vi "_LabeledRectangleDrawTextBackground.vi"(6 "TextHeigth":i32, 7 "GroupName":string, 8 "error in":errorcluster, 9 "Color":u32(colorbox)=16711680, 10 "BoundingBox":T1, 11 "Image Reference In":T3) -> (0 "error out":errorcluster, 3 "Image Reference Out":T3)   [LabVIEW 2020, in "OpenLvVision_Overlays.lvlib"]
uses:
  OpenLvVision_Overlays.lvlib
  <vilib>/OpenLvVision/OpenLvVision_Image/Management/TypeDef/OLV Image.ctl
  TypeDefs/RotatedRectangle.ctl
  TypeDefs/PointI32.ctl
  TypeDefs/DrawingMode.ctl
  TypeDefs/Line.ctl
  <vilib>/OpenLvVision/OpenLvVision_Image/Management/OLV Management.lvlib
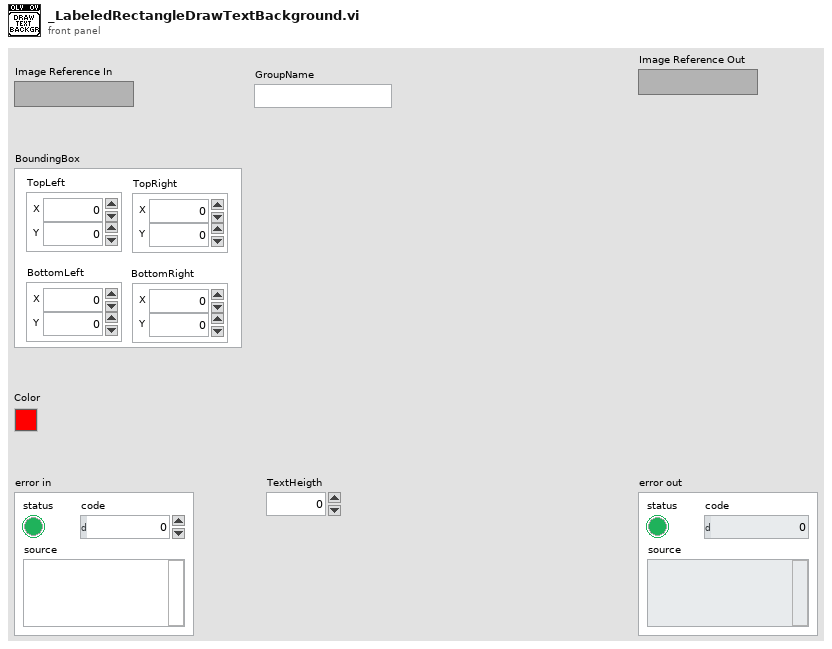
[diagram p1: front panel]
types:
  T1 = typedef "OpenLvVision_Overlays.lvlib/RotatedRectangle.ctl" = cluster{"TopLeft":T2, "TopRight":T2, "BottomRight":T2, "BottomLeft":T2}
  T2 = typedef "OpenLvVision_Overlays.lvlib/PointI32.ctl" = cluster{"X":i32, "Y":i32}
  T3 = typedef "OLV OpenLvVision_Image.lvlib/OLV Management.lvlib/OLV Image.ctl" = refnum<image>
  T4 = typedef "OpenLvVision_Overlays.lvlib/DrawingMode.ctl" = enum16{"Frame", "Fill"}
  T5 = typedef "OpenLvVision_Overlays.lvlib/Line.ctl" = cluster{"StartPoint":T2, "EndPoint":T2}
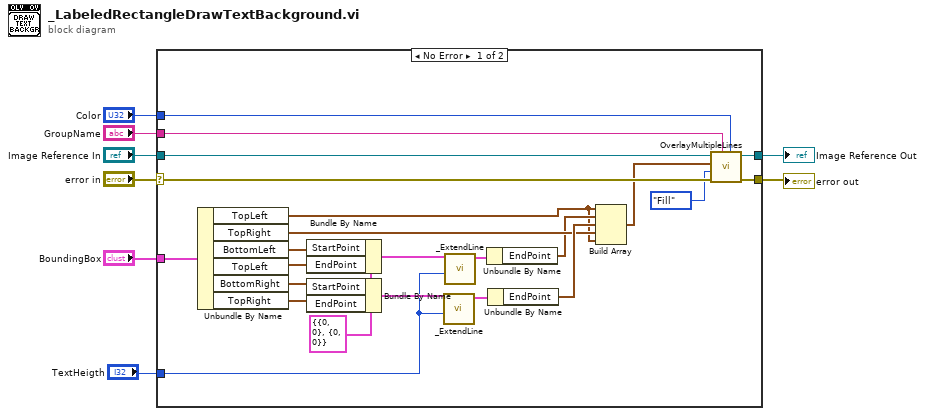
[diagram p0: block diagram]
diagram:
  n1 = case shown="No Error" "error in" {
    selector: "error in" -> [w28 w32]
    tunnel: [w30 w32] -> w7
    tunnel: "Image Reference In" -> [w29 w33]
    tunnel: [w31 w33] -> w6
    tunnel: "GroupName" -> [w27 _]
    tunnel: "Color" -> [w26 _]
    tunnel: "BoundingBox" -> [w25 _]
    tunnel: "TextHeigth" -> [w9 _]
    frame No Error {
      w22 = T5 {"StartPoint"={"X"=0, "Y"=0}, "EndPoint"={"X"=0, "Y"=0}} ("Line")
      n2 = Unbundle By Name(w25) -> ("TopLeft"=w10:T2, "TopRight"=w13:T2, "BottomLeft"=w20:T2, "TopLeft"=w19:T2, "BottomRight"=w18:T2, "TopRight"=w17:T2)
      n3 = Bundle By Name(cluster=w22, "StartPoint"=w20, "EndPoint"=w19) -> (w23:T5)
      n4 = Bundle By Name(cluster=w22, "StartPoint"=w18, "EndPoint"=w17) -> (w21:T5)
      n5 = call "_ExtendLine.vi"("ExtendEnd"=w9, "Line"=w21) -> ("Line"=w15:T5)  [unwired: 9 in]
      n6 = call "_ExtendLine.vi"("ExtendEnd"=w9, "Line"=w23) -> ("Line"=w16:T5)  [unwired: 9 in]
      n7 = Unbundle By Name(w16) -> ("EndPoint"=w12:T2)
      n8 = Unbundle By Name(w15) -> ("EndPoint"=w14:T2)
      n9 = Build Array(w10, w12, w14, w13, w10) -> (w11:T2[])
      n10 = call "OverlayMultipleLines.vi"("Color"=w26, "GroupName"=w27, "error in"=w28, "Drawing Mode (Frame)"=DrawingMode."Fill", "Points"=w11, "Image Reference In"=w29) -> ("error out"=w30:errorcluster, "Image Reference Out"=w31:T3)  [unwired: 4 in]
    }
    frame Error {
    }
  }
  "error out" <- w7
  "Image Reference Out" <- w6
